vi "CSE ISP - error navigation.vi"(7 "Str Refnum":refnum<vi>, 8 "error in":errorcluster, 11 "CSE RefNum":T1) -> (0 "error out":errorcluster)   [LabVIEW 2021]
doc: "::: CalcExpress Toolkit :::\nCopyright (c) 2000-2026 Konstantin Shifershteyn. All rights reserved."
uses:
  vi.lib/addons/CalcExpress/cse.llb/CSE Instance RefNum.ctl
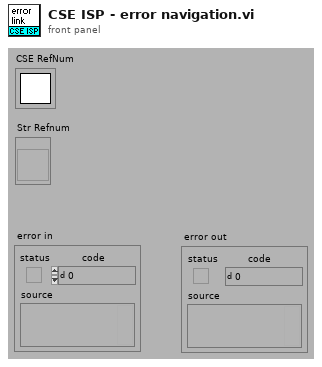
[diagram p1: front panel]
types:
  T1 = typedef "CSE Instance RefNum.ctl" = refnum<k1>
  T2 = typedef "CalcExpress Instance RefNum.ctl" = refnum<k1>
  T3 = cluster{"CE InstanceRef":T2, "post action":enum32{"jump", "jump if true", "jump if false", "stop"}, "jump index":i32, "stmType":i32, "nesting level":i32, "stmOffset":i32, "stmLength":i32, "stmLine ":i32, "expOffset":i32, "expLength":i32, "expLine":i32, "parent index":i32}
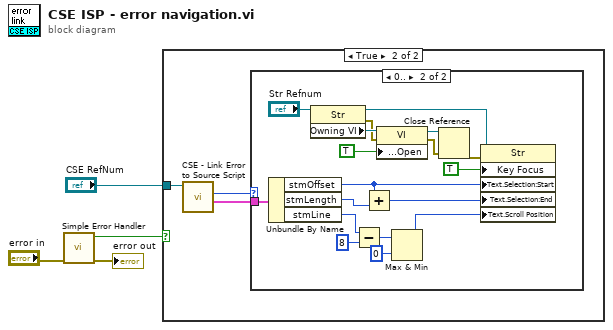
[diagram p0: block diagram]
diagram:
  n1 = call <vilib>:"Simple Error Handler.vi"("error in (no error)"="error in") -> ("error?"=w3:bool, "error out"=→"error out":errorcluster)  [unwired: 4 in, 3 out]
  n2 = case shown="True" w3 {
    tunnel: "CSE RefNum" -> [_ w7]
    frame False {
    }
    frame True {
      n3 = call "CSE - Link Error to Source Script.vi"("CSE RefNum"=w7) -> ("statement info"=w6:T3, "Stm Index"=w5:i32)  [unwired: 4 in, 5 out]
      n4 = case shown="0.." w5 {
        tunnel: w6 -> [_ w25]
        frame ..-1 {
        }
        frame 0.. {
          n5 = Unbundle By Name(w25) -> ("stmOffset"=w23:i32, "stmLength"=w22:i32, "stmLine"=w20:i32)
          n6 = property class="Str"(reference="Str Refnum") -> (reference out=w11:refnum<vi>, error out=w9:errorcluster, "Owning VI"=w13:refnum<vi>)  [unwired: 1 in]
          n7 = Subtract(x=w20, y=8) -> (x-y=w19:i32)
          n8 = Add(x=w23, y=w22) -> (x+y=w24:i32)
          n9 = property class="VI"(reference=w13, error in=w9, "Front Panel Window:Open"=TRUE) -> (reference out=w15:refnum<vi>, error out=w8:errorcluster)
          n10 = Max & Min(x=w19, y=0) -> (max(x,y)=w16:i32)  [unwired: 1 out]
          n11 = Close Reference(reference=w15, error in (no error)=w8) -> (error out=w10:errorcluster)
          n12 = property class="Str"(reference=w11, error in=w10, "Key Focus"=TRUE, "Text.Selection:Start"=w23, "Text.Selection:End"=w24, "Text.Scroll Position"=w16) -> ()  [unwired: 2 out]
        }
      }
    }
  }
